vi "Query Current Angle.vi"(8 "error in (no error)":errorcluster, 11 "CO3000 in":refnum<class "CO3000.lvclass">) -> (0 "error out":errorcluster, 2 "Current Angle":dbl, 3 "CO3000 out":refnum<class "CO3000.lvclass">)   [LabVIEW 2023, in "Turn Table and Mast.lvlib" / "CO3000.lvclass"]
uses:
  CO3000.lvclass
  CO3000.lvclass/CO3000.ctl
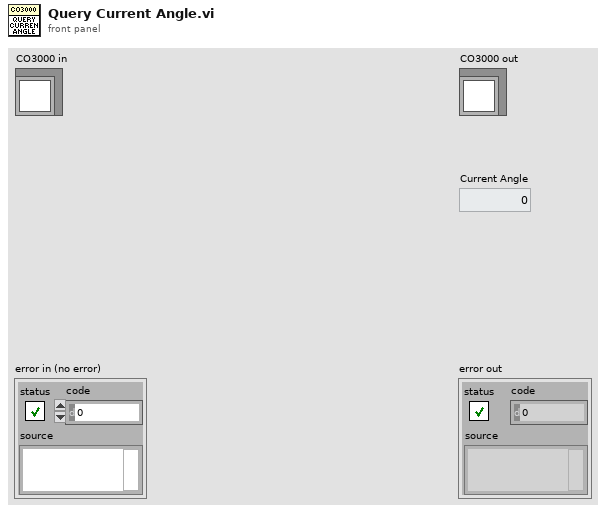
[diagram p1: front panel]
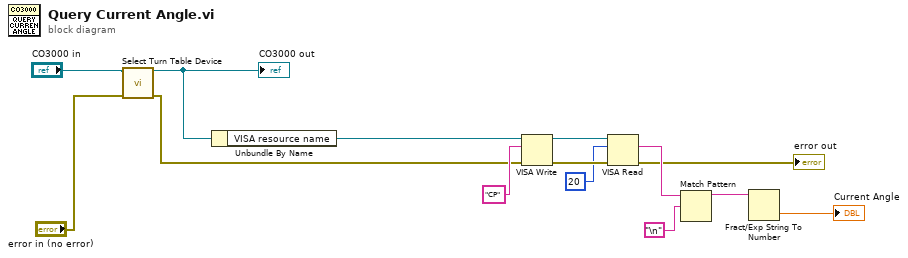
[diagram p0: block diagram]
diagram:
  n1 = call "Select Turn Table Device.vi"("error in (no error)"="error in (no error)", "CO3000 in"="CO3000 in") -> ("error out"=w1:errorcluster, "CO3000 out"=w3:refnum<class "CO3000.lvclass">)  [unwired: 8 in]
  "CO3000 out" <- w3
  n2 = Unbundle By Name(w3) -> ("VISA resource name"=w14:refnum<visa-resource-name>)
  n3 = VISA Write(VISA resource name=w14, write buffer="CP", error in (no error)=w1) -> (VISA resource name out=w12:refnum<visa-resource-name>, error out=w11:errorcluster)  [unwired: 1 out]
  n4 = VISA Read(VISA resource name=w12, byte count=u32 20, error in (no error)=w11) -> (read buffer=w9:string, error out=→"error out":errorcluster)  [unwired: 2 out]
  n5 = Match Pattern(string=w9, regular expression="\n") -> (before substring=w7:string)  [unwired: 1 in, 3 out]
  n6 = Fract/Exp String To Number(string=w7) -> (number=→"Current Angle":dbl)  [unwired: 3 in, 1 out]
